vi "[ce] Normalize Writer IDs to Display History.vi"(10 "size":i32, 11 "writer IDs in":u32[](array[numeric])) -> (2 "disable":u8, 3 "writer IDs":u32[](array[numeric]))   [LabVIEW 2021]
doc: "::: CalcExpress Toolkit :::\nCopyright (c) 2000-2026 Konstantin Shifershteyn. All rights reserved."
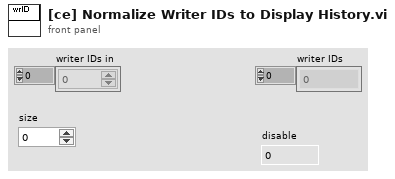
[diagram p1: front panel]
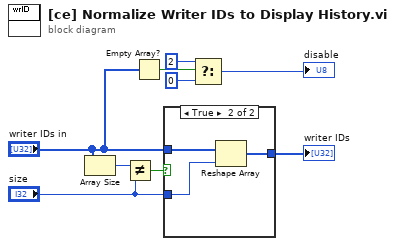
[diagram p0: block diagram]
diagram:
  n1 = Array Size(array="writer IDs in") -> (size(s)=w8:i32)
  n2 = Not Equal?(x=w8, y="size") -> (x != y?=w6:bool)
  n3 = Empty Array?(array="writer IDs in") -> (empty?=w4:bool)
  n4 = case shown="True" w6 {
    tunnel: [w10 w13] -> w9
    tunnel: "writer IDs in" -> [w10 w12]
    tunnel: "size" -> [_ w11]
    frame False {
    }
    frame True {
      n5 = Reshape Array(w12, w11) -> (w13:u32[])
    }
  }
  "writer IDs" <- w9
  n6 = Select(t=u8 2, s=w4, f=u8 0) -> (s? t:f=→"disable":u8)
